vi "Event Catalogue.vi"() -> (0 "corporate actions":T1[](array[typedef]), 1 "earnings":T1[](array[typedef]), 2 "bad news":T1[](array[typedef]), 3 "good news":T1[](array[typedef]))   [LabVIEW 2020, in "Full Featured MCP Server.lvlib"]
doc: "The news that can hit the market at random, as data. Each event has a headline ({stock}, {other} and {sector} are filled in), a scope (one stock, two stocks, the sector of the stock, or the whole market), the direction shown in the news, the immediate jump and the follow: a move of that size that builds up over the next minutes. Jump and follow are log returns (0.05 is about 5 percent); jump other and follow other apply to the second stock. A follow against the jump is an overreaction that partly recovers."
uses:
  Full Featured MCP Server.lvlib
  Event Template.ctl
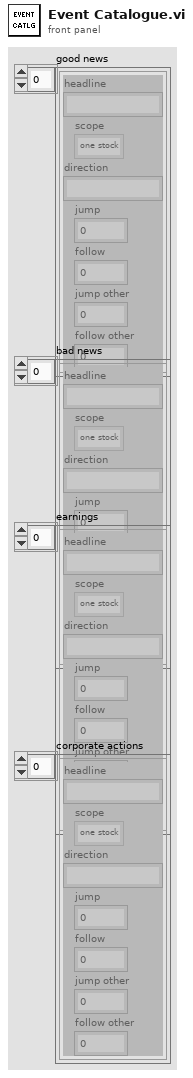
[diagram p1: front panel]
types:
  T1 = typedef "Full Featured MCP Server.lvlib/Event Template.ctl" = cluster{"headline":string, "scope":enum16{"one stock", "two stocks", "sector", "market"}, "direction":string, "jump":dbl, "follow":dbl, "jump other":dbl, "follow other":dbl}
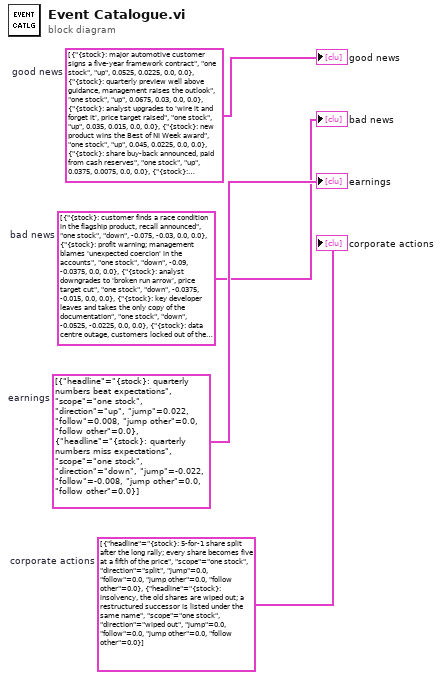
[diagram p0: block diagram]
diagram:
  w4 = T1[] [{"headline"="{stock}: 5-for-1 share split after the long rally; every share becomes five at a fifth of the price", "scope"=enum."one stock", "direction"="split", "jump"=0.0, "follow"=0.0, "jump other"=0.0, "follow other"=0.0}, {"headline"="{stock}: insolvency, the old shares are wiped out; a restructured successor is listed under the same name", "scope"=enum."one stock", "direction"="wiped out", "jump"=0.0, "follow"=0.0, "jump other"=0.0, "follow other"=0.0}]  # corporate actions
  w3 = T1[] [{"headline"="{stock}: quarterly numbers beat expectations", "scope"=enum."one stock", "direction"="up", "jump"=0.022, "follow"=0.008, "jump other"=0.0, "follow other"=0.0}, {"headline"="{stock}: quarterly numbers miss expectations", "scope"=enum."one stock", "direction"="down", "jump"=-0.022, "follow"=-0.008, "jump other"=0.0, "follow other"=0.0}]  # earnings
  w2 = T1[] [{"headline"="{stock}: customer finds a race condition in the flagship product, recall announced", "scope"=enum."one stock", "direction"="down", "jump"=-0.075, "follow"=-0.03, "jump other"=0.0, "follow other"=0.0}, {"headline"="{stock}: profit warning; management blames 'unexpected coercion' in the accounts", "scope"=enum."one stock", "direction"="down", "jump"=-0.09, "follow"=-0.0375, "jump other"=0.0, "follow other"=0.0}, {"headline"="{stock}: analyst downgrades to 'broken run arrow', price target cut", "scope"=enum."one stock", "direction"="down", "jump"=-0.0375, "follow"=-0.015, "jump other"=0.0, "follow other"=0.0}, {"headline"="{stock}: key developer leaves and takes the only copy of the documentation", "scope"=enum."one stock", "direction"="down", "jump"=-0.0525, "follow"=-0.0225, "jump other"=0.0, "follow other"=0.0}, {"headline"="{stock}: data centre outage, customers locked out of their data for a day", "scope"=enum."one stock", "direction"="down", "jump"=-0.0675, "follow"=0.03, "jump other"=0.0, "follow other"=0.0}, {"headline"="{stock}: regulator opens an inquiry into licence server practices", "scope"=enum."one stock", "direction"="down", "jump"=-0.06, "follow"=-0.0375, "jump other"=0.0, "follow other"=0.0}, {"headline"="{stock}: flagship release postponed again, 'next iteration' promised", "scope"=enum."one stock", "direction"="down", "jump"=-0.045, "follow"=-0.0225, "jump other"=0.0, "follow other"=0.0}, {"headline"="{stock}: short-seller report claims revenue was counted twice in a loop", "scope"=enum."one stock", "direction"="down", "jump"=-0.15, "follow"=0.06, "jump other"=0.0, "follow other"=0.0}, {"headline"="{stock}: warehouse fire destroys a quarter's worth of stock", "scope"=enum."one stock", "direction"="down", "jump"=-0.06, "follow"=-0.0075, "jump other"=0.0, "follow other"=0.0}, {"headline"="{stock}: chief executive sells a large block of his own shares 'for personal reasons'", "scope"=enum."one stock", "direction"="down", "jump"=-0.045, "follow"=-0.03, "jump other"=0.0, "follow other"=0.0}, {"headline"="{stock} loses a patent dispute against {other} and must pay licence fees", "scope"=enum."two stocks", "direction"="mixed", "jump"=-0.06, "follow"=-0.0225, "jump other"=0.0375, "follow other"=0.015}, {"headline"="{stock} loses its largest customer to {other}", "scope"=enum."two stocks", "direction"="mixed", "jump"=-0.0825, "follow"=-0.03, "jump other"=0.0525, "follow other"=0.0225}, {"headline"="{sector}: chip shortage delays deliveries across the sector", "scope"=enum."sector", "direction"="down", "jump"=-0.03, "follow"=-0.018, "jump other"=0.0, "follow other"=0.0}, {"headline"="{sector}: big customer freezes budgets, orders across the sector postponed", "scope"=enum."sector", "direction"="down", "jump"=-0.024, "follow"=-0.024, "jump other"=0.0, "follow other"=0.0}, {"headline"="{sector}: security flaw found in a library the whole sector depends on", "scope"=enum."sector", "direction"="down", "jump"=-0.042, "follow"=0.012, "jump other"=0.0, "follow other"=0.0}, {"headline"="Market: interest rate decision postponed; DAQ cards idle", "scope"=enum."market", "direction"="down", "jump"=-0.01, "follow"=-0.007, "jump other"=0.0, "follow other"=0.0}, {"headline"="Market: weak industry outlook, investors pull the stop button", "scope"=enum."market", "direction"="down", "jump"=-0.018, "follow"=-0.01, "jump other"=0.0, "follow other"=0.0}]  # bad news
  w1 = T1[] [{"headline"="{stock}: major automotive customer signs a five-year framework contract", "scope"=enum."one stock", "direction"="up", "jump"=0.0525, "follow"=0.0225, "jump other"=0.0, "follow other"=0.0}, {"headline"="{stock}: quarterly preview well above guidance, management raises the outlook", "scope"=enum."one stock", "direction"="up", "jump"=0.0675, "follow"=0.03, "jump other"=0.0, "follow other"=0.0}, {"headline"="{stock}: analyst upgrades to 'wire it and forget it', price target raised", "scope"=enum."one stock", "direction"="up", "jump"=0.035, "follow"=0.015, "jump other"=0.0, "follow other"=0.0}, {"headline"="{stock}: new product wins the Best of NI Week award", "scope"=enum."one stock", "direction"="up", "jump"=0.045, "follow"=0.0225, "jump other"=0.0, "follow other"=0.0}, {"headline"="{stock}: share buy-back announced, paid from cash reserves", "scope"=enum."one stock", "direction"="up", "jump"=0.0375, "follow"=0.0075, "jump other"=0.0, "follow other"=0.0}, {"headline"="{stock}: long-standing memory leak finally found and fixed, customers return", "scope"=enum."one stock", "direction"="up", "jump"=0.06, "follow"=0.0375, "jump other"=0.0, "follow other"=0.0}, {"headline"="{stock}: surprise licence deal with a large test-system integrator", "scope"=enum."one stock", "direction"="up", "jump"=0.09, "follow"=0.0225, "jump other"=0.0, "follow other"=0.0}, {"headline"="{stock}: takeover rumour sends the shares soaring; the company declines to comment", "scope"=enum."one stock", "direction"="up", "jump"=0.135, "follow"=-0.06, "jump other"=0.0, "follow other"=0.0}, {"headline"="{stock}: certification passed at the first attempt, shipments start early", "scope"=enum."one stock", "direction"="up", "jump"=0.0375, "follow"=0.0225, "jump other"=0.0, "follow other"=0.0}, {"headline"="{stock}: activist investor takes a stake and demands a block diagram clean-up", "scope"=enum."one stock", "direction"="up", "jump"=0.075, "follow"=-0.0225, "jump other"=0.0, "follow other"=0.0}, {"headline"="{stock} poaches the lead architect of {other}", "scope"=enum."two stocks", "direction"="mixed", "jump"=0.045, "follow"=0.015, "jump other"=-0.0375, "follow other"=-0.015}, {"headline"="{stock} wins a benchmark shoot-out against {other}; customers take note", "scope"=enum."two stocks", "direction"="mixed", "jump"=0.0525, "follow"=0.0225, "jump other"=-0.035, "follow other"=-0.015}, {"headline"="{sector}: NI Week keynote calls the sector 'strategic', order books fill", "scope"=enum."sector", "direction"="up", "jump"=0.03, "follow"=0.018, "jump other"=0.0, "follow other"=0.0}, {"headline"="{sector}: government test-lab programme announced, suppliers expect a boost", "scope"=enum."sector", "direction"="up", "jump"=0.024, "follow"=0.024, "jump other"=0.0, "follow other"=0.0}, {"headline"="{sector}: large aerospace project standardises on the sector's tools", "scope"=enum."sector", "direction"="up", "jump"=0.036, "follow"=0.012, "jump other"=0.0, "follow other"=0.0}, {"headline"="Market: surprise interest rate cut; even idle DAQ cards rally", "scope"=enum."market", "direction"="up", "jump"=0.015, "follow"=0.01, "jump other"=0.0, "follow other"=0.0}, {"headline"="Market: strong industry order numbers lift the whole exchange", "scope"=enum."market", "direction"="up", "jump"=0.013, "follow"=0.01, "jump other"=0.0, "follow other"=0.0}]  # good news
  "good news" <- w1
  "bad news" <- w2
  "earnings" <- w3
  "corporate actions" <- w4
